vi "GenerateEventItemBuilt.vi"(9 "ProjectItem":refnum<class "ProjectItem.lvclass">, 10 "Result":string, 11 "ItemBuilt":T1) -> ()   [LabVIEW 2019, in "SolutionBuilder.lvlib" / "ProjectItem.lvclass"]
uses:
  ProjectItem.lvclass
  Events/EventItemBuilt.ctl
  ProjectItem.lvclass/ProjectItem.ctl
  SolutionBuilder.lvlib
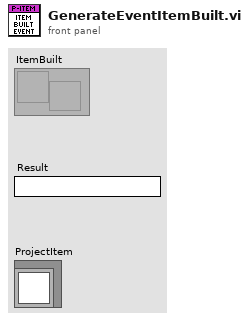
[diagram p1: front panel]
types:
  T1 = typedef "SolutionBuilder.lvlib/EventItemBuilt.ctl" = refnum<user-event>
  T2 = cluster{"Build spec name":string, "Target":string, "Owning lib name":string, "t":string}
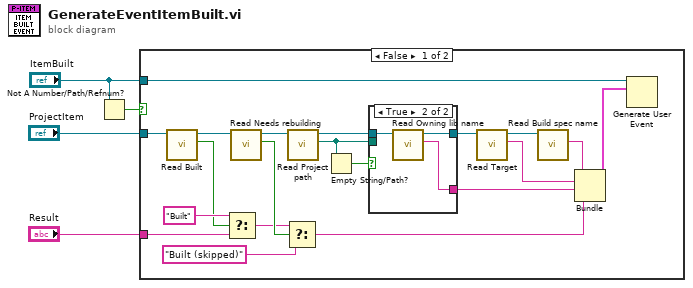
[diagram p0: block diagram]
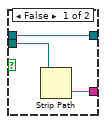
[diagram p2: hidden frame]
diagram:
  n1 = Not A Number/Path/Refnum?(number/path/refnum="ItemBuilt") -> (NaN/Path/Refnum?=w1:bool)
  n2 = case shown="False" w1 {
    tunnel: "ProjectItem" -> [w24 _]
    tunnel: "Result" -> [w20 _]
    tunnel: "ItemBuilt" -> [w19 _]
    frame False {
      n3 = call-dynamic "Read Built.vi"("ProjectItem in"=w24) -> ("Built"=w16:bool, "ProjectItem out"=w10:refnum<class "ProjectItem.lvclass">)  [unwired: 9 in]
      n4 = Select(t="Built" ("name"), s=w16, f=w20) -> (s? t:f=w6:string)
      n5 = call-dynamic "Read Needs rebuilding.vi"("ProjectItem in"=w10) -> ("Needs rebuilding"=w8:bool, "ProjectItem out"=w9:refnum<class "ProjectItem.lvclass">)  [unwired: 9 in]
      n6 = Select(t=w6, s=w8, f="Built (skipped)" ("t")) -> (s? t:f=w7:string)
      n7 = call-dynamic "Read Project path.vi"("ProjectItem in"=w9) -> ("Project path"=w12:path, "ProjectItem out"=w13:refnum<class "ProjectItem.lvclass">)  [unwired: 9 in]
      n8 = Empty String/Path?(string/path=w12) -> (empty?=w11:bool)
      n9 = case shown="True" w11 {
        tunnel: w13 -> [w26 w30]
        tunnel: [w27 w28] -> w14
        tunnel: [w26 w29] -> w15
        tunnel: w12 -> [w25 _]
        frame False {
          n10 = Strip Path(path=w25) -> (name=w27:string)  [unwired: 1 out]
        }
        frame True {
          n11 = call-dynamic "Read Owning lib name.vi"("ProjectItem in"=w30) -> ("Owning lib name"=w28:string, "ProjectItem out"=w29:refnum<class "ProjectItem.lvclass">)  [unwired: 9 in]
        }
      }
      n12 = call "Read Target.vi"("ProjectItem in"=w15) -> ("Target"=w17:string, "ProjectItem out"=w18:refnum<class "ProjectItem.lvclass">)  [unwired: 9 in]
      n13 = call-dynamic "Read Build spec name.vi"("ProjectItem in"=w18) -> ("Build spec name"=w23:string)  [unwired: 9 in, 1 out]
      n14 = Bundle("Build spec name"=w23, "Target"=w17, "Owning lib name"=w14, "t"=w7) -> (w21:T2)  [unwired: 1 in]
      n15 = Generate User Event(user event=w19, event data cluster=w21) -> ()  [unwired: 2 in, 2 out]
    }
    frame True {
    }
  }
